vi "FlyWheelCtrl_Example.vi"() -> ()   [LabVIEW 2019]
uses:
  <vilib>/Rock Robotics/WPI/ThirdParty/JAS_Junk/TrajLib/TypeDef/DCMOTOR.CTL
  <vilib>/Rock Robotics/WPI/ThirdParty/JAS_Junk/TrajLib/TypeDef/LINEAR_SYSTEM.ctl
  <vilib>/Analysis/Matrix/Datatypes/RealMatrix.ctl
  <vilib>/Rock Robotics/WPI/ThirdParty/JAS_Junk/TrajLib/TypeDef/FLYWHEEL_SIM.ctl
  <vilib>/Rock Robotics/WPI/ThirdParty/JAS_Junk/TrajLib/TypeDef/LINEAR_SYSTEM_SIM.ctl
  <vilib>/Rock Robotics/WPI/ThirdParty/JAS_Junk/TrajLib/Enum/DCMOTOR_TYPES_ENUM.ctl
  <vilib>/Rock Robotics/WPI/ThirdParty/JAS_Junk/TrajLib/LinearFilter_LP_BW2_Execute.vi
  <vilib>/Rock Robotics/WPI/ThirdParty/JAS_Junk/TrajLib/VI/BoolCmd_Send_Internal.vi
  <vilib>/Rock Robotics/WPI/ThirdParty/JAS_Junk/TrajLib/VI/numCmd_ObtainQueue_OneDbl.vi
  <vilib>/Rock Robotics/WPI/ThirdParty/JAS_Junk/TrajLib/VI/BoolCmd_Recv_Internal.vi
  <vilib>/Rock Robotics/WPI/ThirdParty/JAS_Junk/TrajLib/LinearFilter_ResetToValue.vi
  <vilib>/Rock Robotics/WPI/ThirdParty/JAS_Junk/TrajLib/LinearFilter_Calculate.vi
  <vilib>/Rock Robotics/WPI/ThirdParty/JAS_Junk/TrajLib/VI/BoolCmd_ObtainQueue.vi
  <vilib>/Rock Robotics/WPI/ThirdParty/JAS_Junk/TrajLib/LinearFilter_LowPassBW2.vi
  <vilib>/Rock Robotics/WPI/ThirdParty/JAS_Junk/TrajLib/Trajectory_Library.lvlib
  <vilib>/Analysis/Matrix/NI_Matrix.lvlib
panel:
  in  "Tab Control":T1(tab)
  in  "Speed Setpoint RPM":dbl=2500.0 format="%20.3f"
  out "Motor Current":dbl format="%20.3f"
  out "Battery \nVoltage":dbl format="%20.3f"
  in  "Shoot ball":bool
  out "CO Chart":T2(graph)
  in  "Shooter On/Off":bool
  out "Encoer Speed\nRPM":dbl(slide) scale=0.0..5500.0
  out "Speed RPM":dbl format="%20.3f"
  out "Kalman Filtered\nSpeed RPM":dbl format="%20.3f"
  out "PV Chart":T3(graph)
  out "Controller Error":bool
  out "Motor Volt Dmd (CO)":dbl format="%20.3f"
  out "shoot Start":bool
  out "Shoot Done":bool
  out "Shooter Motor":T4 {"Jr_KgM2" format="%13.5p"; "L_H" format="%13.5p"; "Kt_NMPerAmp" format="%13.5p"; "KvINV_RadPerSecPerVolt" format="%13.5p"; "R_Ohms" format="%13.5p"; "FreeSpeed_RadPerSec" format="%13.5p"; "FreeCurrent_Amps" format="%13.5p"; "StallCurrent_Amps" format="%13.5p"; "StallTorque_NM" format="%13.5p"; "nominalVoltage_Volts" format="%13.5p"}
  out "m_flywheelPlant":T5
  out "m_FlyWheelSim":T7 {"GearBox"."Jr_KgM2" format="%13.5p"; "GearBox"."L_H" format="%13.5p"; "GearBox"."Kt_NMPerAmp" format="%13.5p"; "GearBox"."KvINV_RadPerSecPerVolt" format="%13.5p"; "GearBox"."R_Ohms" format="%13.5p"; "GearBox"."FreeSpeed_RadPerSec" format="%13.5p"; "GearBox"."FreeCurrent_Amps" format="%13.5p"; "GearBox"."StallCurrent_Amps" format="%13.5p"; "GearBox"."StallTorque_NM" format="%13.5p"; "GearBox"."nominalVoltage_Volts" format="%13.5p"}
  out "Shooting A":T6
  out "Shooting B":T6
  # "<States,States>"
  # "<States,Inputs>"
  # "<Outputs,States>"
  # "<Outputs,Inputs>"
  # "<States, 1>"
  # "<Outputs, 1>"
  # "<Inputs, 1>"
  # "<Outputs, 1>"
  # "<States,States>"
  # "<States,Inputs>"
  # "<Outputs,States>"
  # "<Outputs,Inputs>"
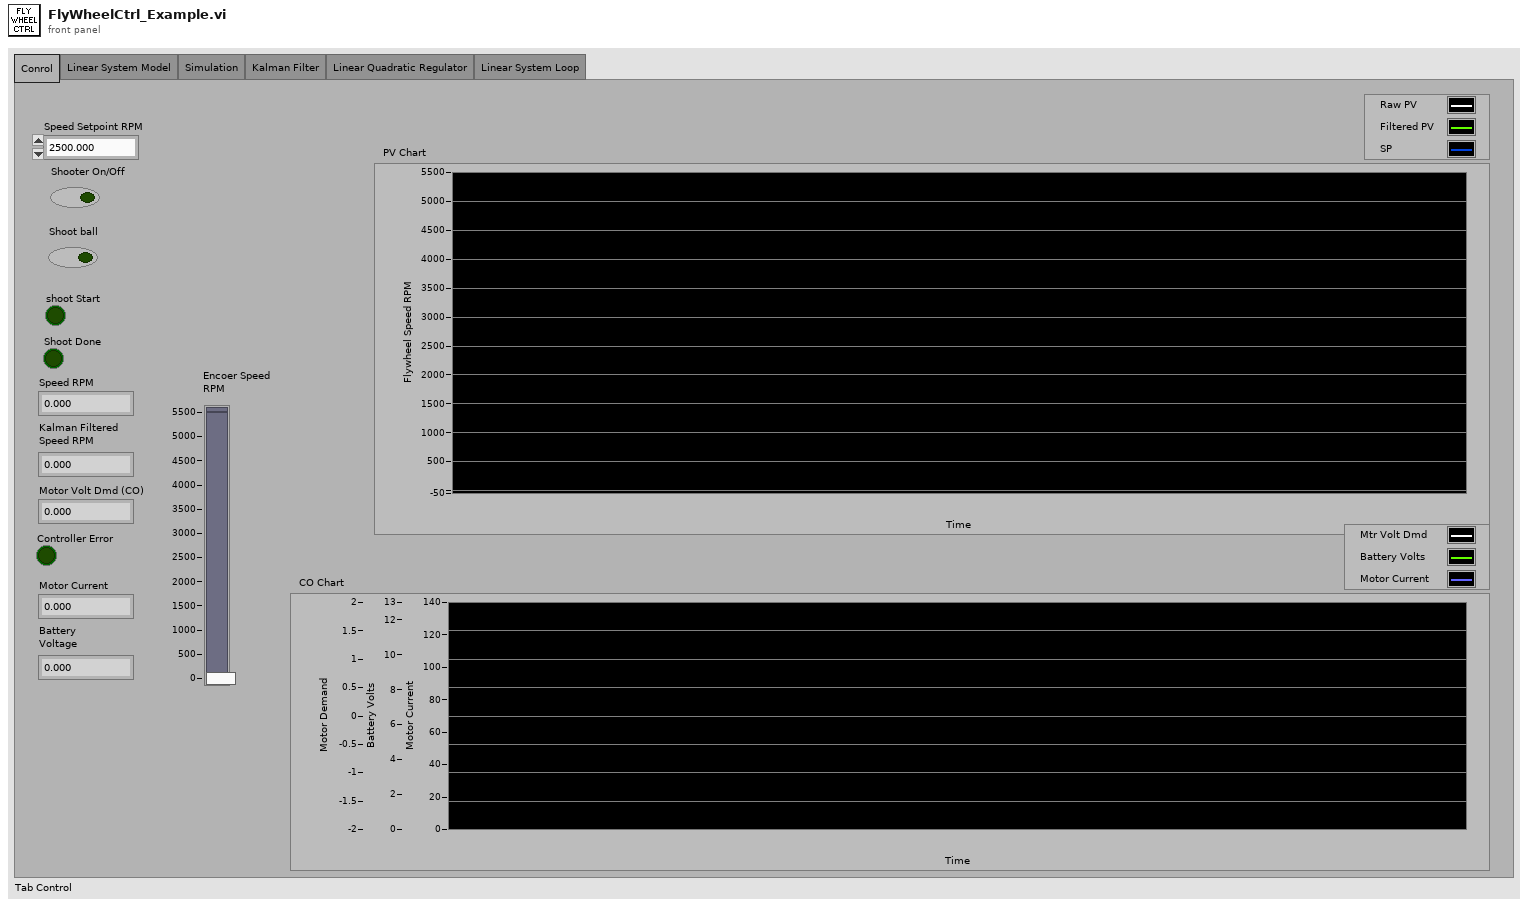
[diagram p1: front panel]
types:
  T1 = enum32{"Conrol", "Linear System Model", "Simulation", "Kalman Filter", "Linear Quadratic Regulator", "Linear System Loop"}
  T2 = cluster{"f":dbl, "Voltage":dbl, "Motor Current":dbl}
  T3 = cluster{"upper limit":dbl, "Real Matrix Element":dbl, "Real Matrix Element":dbl}
  T4 = typedef "Trajectory_Library.lvlib/DCMOTOR.CTL" = cluster{"nominalVoltage_Volts":dbl, "StallTorque_NM":dbl, "StallCurrent_Amps":dbl, "FreeCurrent_Amps":dbl, "FreeSpeed_RadPerSec":dbl, "R_Ohms":dbl, "KvINV_RadPerSecPerVolt":dbl, "Kt_NMPerAmp":dbl, "L_H":dbl, "Jr_KgM2":dbl}
  T5 = typedef "Trajectory_Library.lvlib/LINEAR_SYSTEM.ctl" = cluster{"m_A":T6, "m_B":T6, "m_C":T6, "m_D":T6, "States":i32, "Inputs":i32, "Outputs":i32}
  T6 = typedef "NI_Matrix.lvlib/RealMatrix.ctl" = dbl[][]
  T7 = typedef "Trajectory_Library.lvlib/FLYWHEEL_SIM.ctl" = cluster{"LinearSystemSim":T8, "GearBox":T4, "Gearing":dbl}
  T8 = typedef "Trajectory_Library.lvlib/LINEAR_SYSTEM_SIM.ctl" = cluster{"m_Plant":T5, "m_X":T6, "m_Y":T6, "m_U":T6, "MeasureStdDev":T6}
  T9 = cluster{"RotationsPerMinute":dbl, "Value":dbl, "Value":dbl}
  T10 = typedef "Trajectory_Library.lvlib/DCMOTOR_TYPES_ENUM.ctl" = enum16{"CIM", "AndyMark 9015", "Andy Mark RS 775 125", "Bag", "BaneBots RS 550", "BaneBots RS 775", "Falcon 500", "Mini CIM", "NEO", "NEO 550", "Romi BuiltIn", "Vex 775 Pro", "Snow Blower AM 2235A", "Bosch Seat AM 3493", "Falcon 500 FOC", "Kraken X60", "Kraken X60 FOC", "NEO Vortex"}
  T11 = typedef "Trajectory_Library.lvlib/LINEAR_SYSTEM_ID_FLYWHEEL_MODEL.ctl" = cluster{"DCMOTOR_TYPES":T10, "Num Motors":i32, "Gearing":dbl, "MOI kgm2":dbl}
  T12 = typedef "Trajectory_Library.lvlib/LINEAR_SYSTEM_LOOP_FLYWHEEL_CTRL_PARAMS.CTL" = cluster{"Vel Model Std Dev Rad/Sec":dbl, "Vel Meas Std Dev Rad/Sec":dbl, "Vel Ctrl Tol Rad/Sec":dbl, "Max Ctrl Out V":dbl}
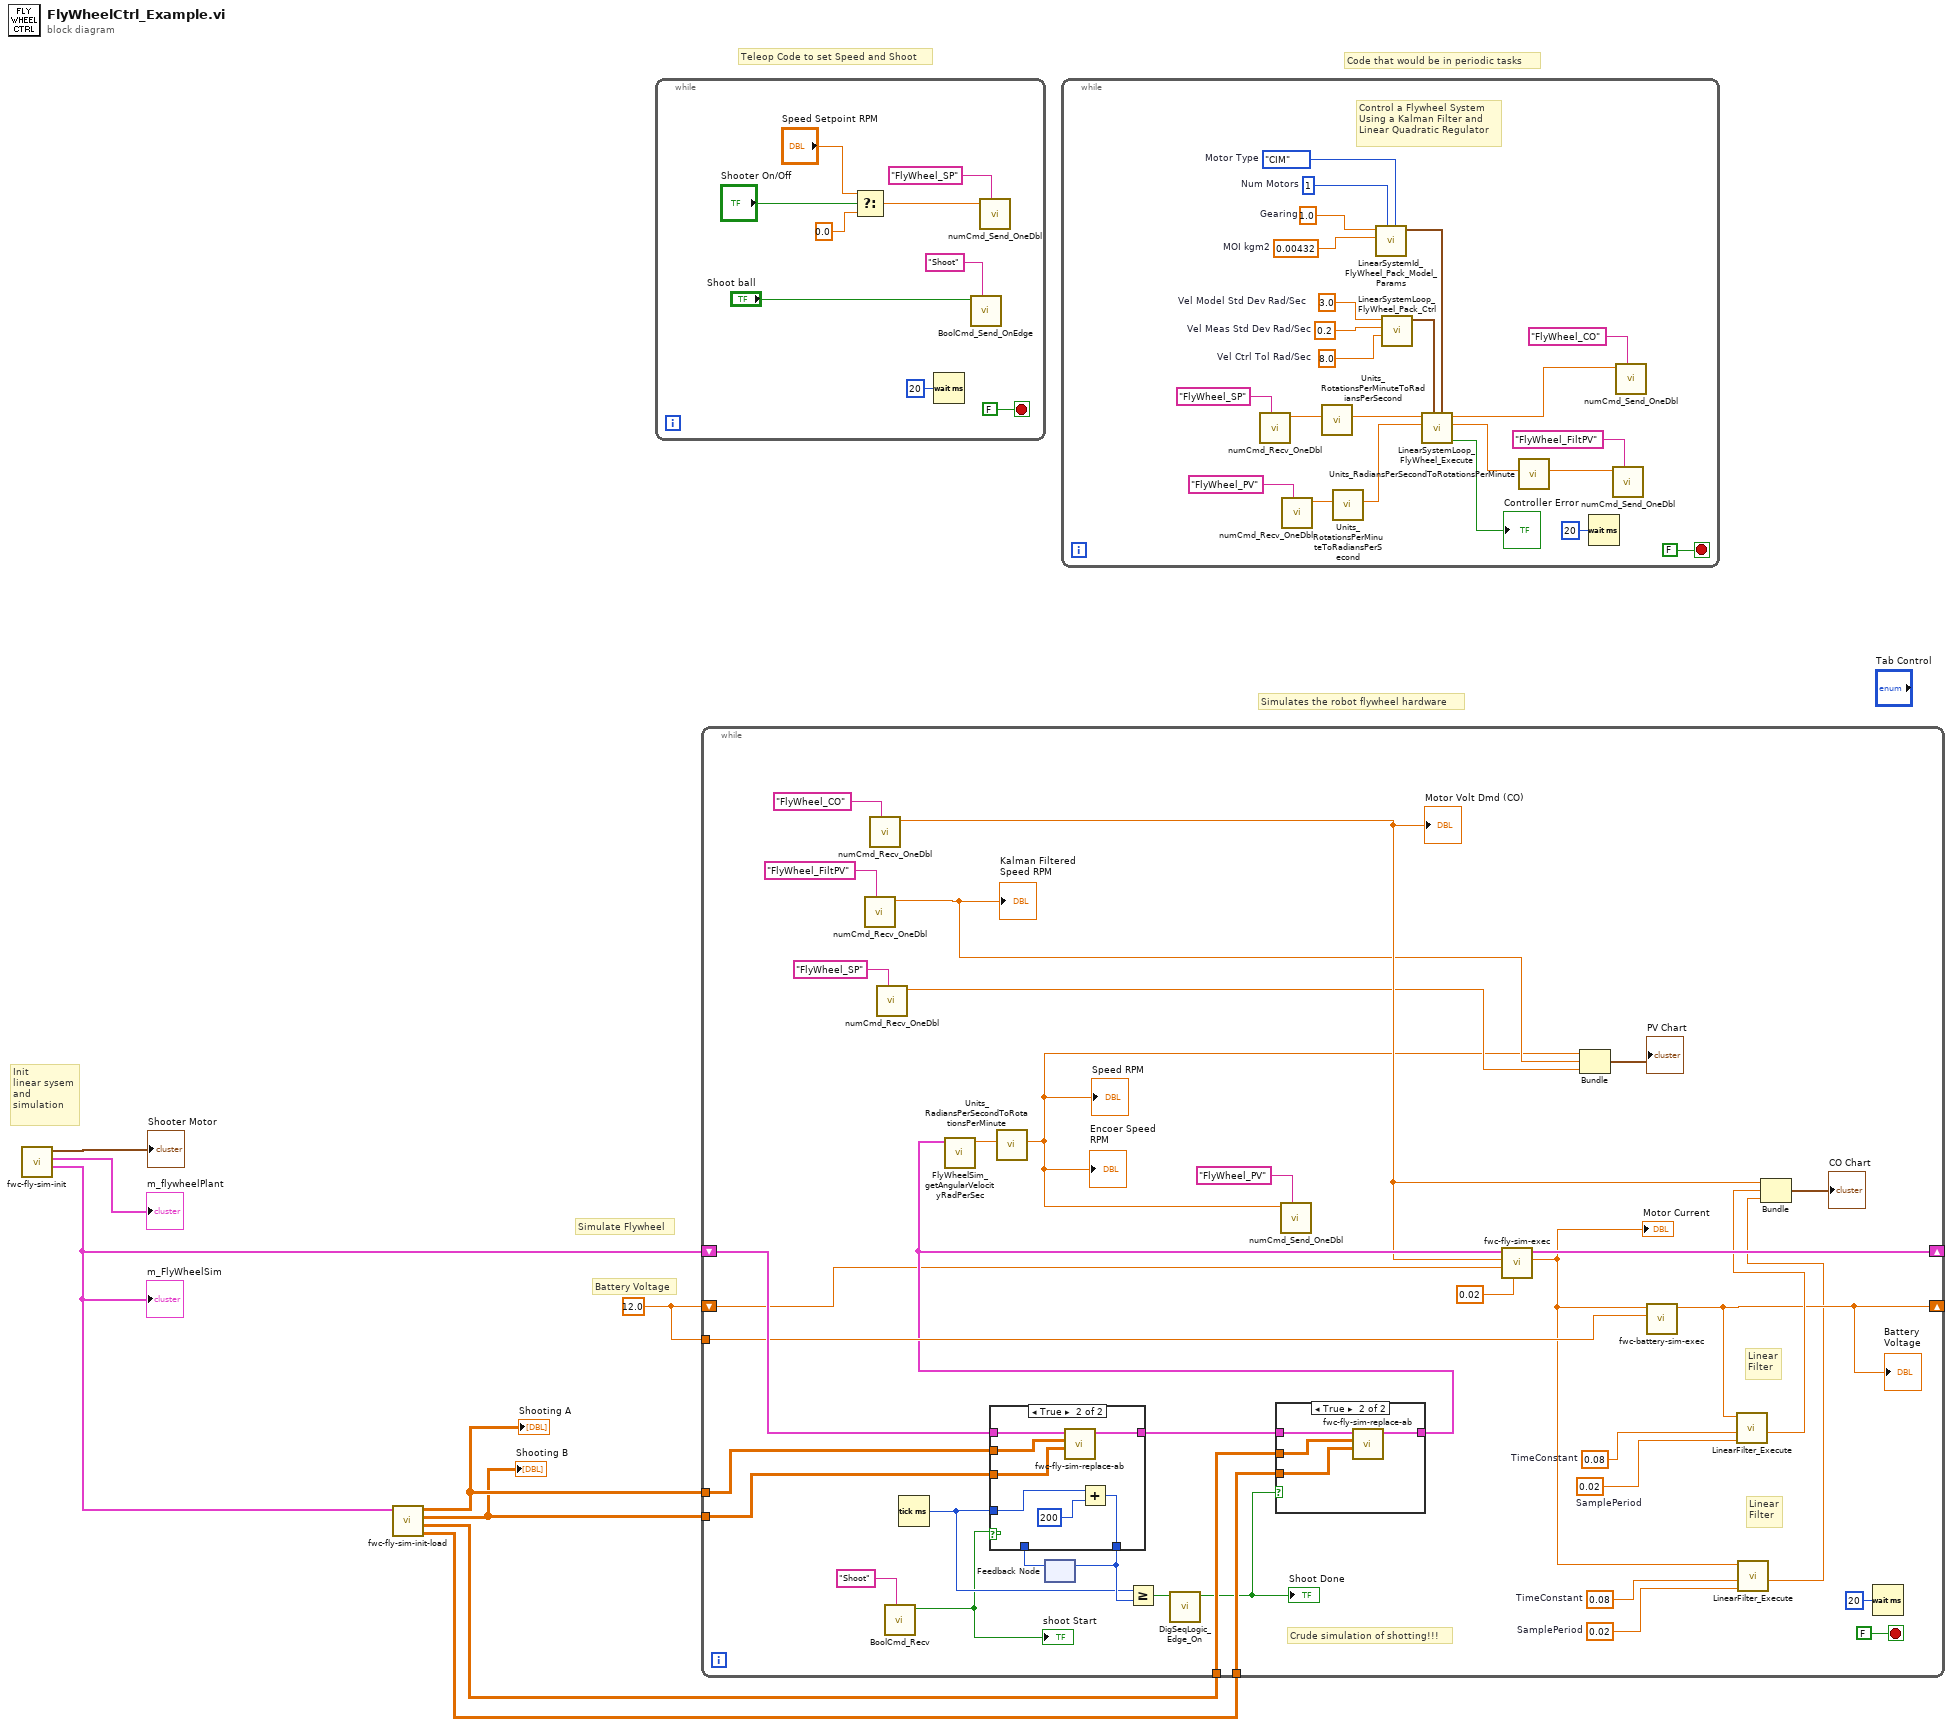
[diagram p0: block diagram]
diagram:
  w7 = 12.0
  # "Teleop Code to set Speed and Shoot"
  # "Code that would be in periodic tasks"
  # "Simulates the robot flywheel hardware"
  # "Init\nlinear sysem\nand \nsimulation"
  # "Simulate Flywheel"
  # "Battery Voltage"
  n1 = call "fwc-fly-sim-init.vi"() -> ("FlyWheelSim"=w6:T7, "Linearsystem"=→"m_flywheelPlant":T5, "DCMOTOR"=→"Shooter Motor":T4)  [unwired: 9 in]
  "m_FlyWheelSim" <- w6
  n2 = call "fwc-fly-sim-init-load.vi"("FlyWheelSim"=w6) -> ("Normal B"=w1:T6, "Normal A"=w2:T6, "Loaded B"=w4:T6, "Loaded A"=w5:T6)  [unwired: 7 in]
  "Shooting A" <- w5
  "Shooting B" <- w4
  n3 = while {
    stop <- FALSE stop-if-true
    n4 = Select(t="Speed Setpoint RPM", s="Shooter On/Off", f=0.0) -> (s? t:f=w14:dbl)
    n5 = Wait (ms)(milliseconds to wait=u32 20) -> ()  [unwired: 1 out]
    n6 = call <vilib>:"BoolCmd_Send_OnEdge.vi"("Command Name"="Shoot", "Value"="Shoot ball") -> ()  [unwired: 9 in, 1 out]
    n7 = call <vilib>:"numCmd_Send_OneDbl.vi"("Command Name"="FlyWheel_SP", "Value"=w14) -> ()  [unwired: 9 in, 1 out]
  }
  n8 = while {
    shift-right: [w53] -> _
    shift-left: w6 -> [w51]
    shift-right: [w35] -> _
    shift-left: w7 -> [w39]
    tunnel: w7 -> [w43]
    tunnel: w2 -> [w49]
    tunnel: w1 -> [w48]
    tunnel: w5 -> [w47]
    tunnel: w4 -> [w46]
    stop <- FALSE stop-if-true
    w37 = 0.02  # SamplePeriod
    w19 = 0.08  # TimeConstant
    w38 = 0.02  # SamplePeriod
    w18 = 0.08  # TimeConstant
    # "Linear\nFilter"
    # "Linear\nFilter"
    # "Crude simulation of shotting!!!"
    n9 = call <vilib>:"numCmd_Recv_OneDbl.vi"("Command Name"="FlyWheel_FiltPV") -> ("Value"=w29:dbl)  [unwired: 8 in, 2 out]
    "Kalman Filtered\nSpeed RPM" <- w29
    n10 = call <vilib>:"numCmd_Recv_OneDbl.vi"("Command Name"="FlyWheel_CO") -> ("Value"=w31:dbl)  [unwired: 8 in, 2 out]
    "Motor Volt Dmd (CO)" <- w31
    n11 = call <vilib>:"numCmd_Recv_OneDbl.vi"("Command Name"="FlyWheel_SP") -> ("Value"=w27:dbl)  [unwired: 8 in, 2 out]
    n12 = call <vilib>:"BoolCmd_Recv.vi"("Command Name"="Shoot") -> ("New Request"=w20:bool)  [unwired: 9 in, 1 out]
    "shoot Start" <- w20
    n13 = Tick Count (ms)() -> (millisecond timer value=w42:u32)
    n14 = feedback #1() -> (w44:u32)  [unwired: 1 in]
    n15 = case shown="True" w20 {
      tunnel: w51 -> [w63 w68]
      tunnel: [w63 w67] -> w50
      tunnel: w47 -> [_ w66]
      tunnel: w46 -> [_ w65]
      tunnel: [w62 w69] -> w45
      tunnel: w44 -> [w62 _]
      tunnel: w42 -> [_ w64]
      frame False {
      }
      frame True {
        n16 = call "fwc-fly-sim-replace-ab.vi"("B"=w65, "A"=w66, "in FlyWheelSim"=w68) -> ("out FlyWheelSim"=w67:T7)  [unwired: 8 in]
        n17 = Add(x=w64, y=u32 200) -> (x+y=w69:u32)
      }
    }
    n18 = feedback-in #1(w45) -> ()
    n19 = Greater Or Equal?(x=w42, y=w45) -> (x >= y?=w22:bool)
    n20 = call <vilib>:"DigSeqLogic_Edge_On.vi"("Input"=w22) -> ("On Edge"=w23:bool)  [unwired: 10 in]
    "Shoot Done" <- w23
    n21 = case shown="True" w23 {
      tunnel: w50 -> [w57 w61]
      tunnel: [w57 w60] -> w40
      tunnel: w49 -> [_ w59]
      tunnel: w48 -> [_ w58]
      frame False {
      }
      frame True {
        n22 = call "fwc-fly-sim-replace-ab.vi"("B"=w58, "A"=w59, "in FlyWheelSim"=w61) -> ("out FlyWheelSim"=w60:T7)  [unwired: 8 in]
      }
    }
    n23 = call <vilib>:"FlyWheelSim_getAngularVelocityRadPerSec.vi"("FlyWheelSim"=w40) -> ("Velocity_RadPerSec"=w26:dbl)  [unwired: 10 in]
    n24 = call <vilib>:"Units_RadiansPerSecondToRotationsPerMinute.vi"("RadiansPerSecond"=w26) -> ("RotationsPerMinute"=w24:dbl)  [unwired: 10 in]
    "Encoer Speed\nRPM" <- w24
    "Speed RPM" <- w24
    n25 = call <vilib>:"numCmd_Send_OneDbl.vi"("Command Name"="FlyWheel_PV", "Value"=w24) -> ()  [unwired: 9 in, 1 out]
    n26 = call "fwc-fly-sim-exec.vi"("dT_Seconds"=0.02, "Battery Voltage"=w39, "Motor Dmd (CO)"=w31, "in FlyWheelSim"=w40) -> ("Motor Current"=w34:dbl, "out FlyWheelSim"=w53:T7)  [unwired: 6 in]
    "Motor Current" <- w34
    n27 = Bundle("RotationsPerMinute"=w24, "Value"=w29, "Value"=w27) -> (→"PV Chart":T9)  [unwired: 1 in]
    n28 = call "fwc-battery-sim-exec.vi"("Numeric"=w43, "Motor Current"=w34) -> ("Voltage"=w35:dbl)  [unwired: 9 in]
    "Battery \nVoltage" <- w35
    n29 = call-poly <vilib>:"LinearFilter_Execute.vi"("SamplePeriod"=w38, "TimeConstant"=w18, "Input"=w35) -> ("Output"=w36:dbl)  [unwired: 8 in]
    n30 = call-poly <vilib>:"LinearFilter_Execute.vi"("SamplePeriod"=w37, "TimeConstant"=w19, "Input"=w34) -> ("Output"=w33:dbl)  [unwired: 8 in]
    n31 = Bundle("Value"=w31, "Output"=w36, "Output"=w33) -> (→"CO Chart":cluster{"Value":dbl, "Output":dbl, "Output":dbl})  [unwired: 1 in]
    n32 = Wait (ms)(milliseconds to wait=u32 20) -> ()  [unwired: 1 out]
  }
  n33 = while {
    stop <- FALSE stop-if-true
    w83 = 3.0  # Vel Model Std Dev Rad/Sec
    w84 = 0.2  # Vel Meas Std Dev Rad/Sec
    w85 = 8.0  # Vel Ctrl Tol Rad/Sec
    w90 = 1.0  # Gearing
    w91 = 0.00432  # MOI kgm2
    w92 = 1  # Num Motors
    w93 = DCMOTOR_TYPES_ENUM."CIM"  # Motor Type
    # "Control a Flywheel System\nUsing a Kalman Filter and \nLinear Quadratic Regulator"
    n34 = call <vilib>:"numCmd_Recv_OneDbl.vi"("Command Name"="FlyWheel_SP") -> ("Value"=w77:dbl)  [unwired: 8 in, 2 out]
    n35 = call <vilib>:"numCmd_Recv_OneDbl.vi"("Command Name"="FlyWheel_PV") -> ("Value"=w81:dbl)  [unwired: 8 in, 2 out]
    n36 = call <vilib>:"Units_RotationsPerMinuteToRadiansPerSecond.vi"("RotationsPerMinute"=w77) -> ("RadiansPerSecond"=w79:dbl)  [unwired: 10 in]
    n37 = call <vilib>:"Units_RotationsPerMinuteToRadiansPerSecond.vi"("RotationsPerMinute"=w81) -> ("RadiansPerSecond"=w80:dbl)  [unwired: 10 in]
    n38 = call <vilib>:"LinearSystemId_FlyWheel_Pack_Model_Params.vi"("DCMOTOR_TYPES"=w93, "Num Motors"=w92, "MOI kgm2"=w91, "Gearing"=w90) -> ("LinearSystem_ID_FlyWheel_Model"=w87:T11)  [unwired: 7 in]
    n39 = call <vilib>:"LinearSystemLoop_FlyWheel_Pack_Ctrl.vi"("Vel Ctrl Tol Rad/Sec"=w85, "Vel Meas Std Dev Rad/Sec"=w84, "Vel Model Std Dev Rad/Sec"=w83) -> ("LinearSystemLoop_FlyWheel_Ctrl_Params"=w86:T12)  [unwired: 8 in]
    n40 = call <vilib>:"LinearSystemLoop_FlyWheel_Execute.vi"("FlyWheelSim_Model _Params"=w87, "LinearSystem_FlyWheel_Ctrl_Params"=w86, "Velocity (Rad/Sec)\n(PV)"=w80, "Velocity (Rad/Sec)\nSetpoint (SP)"=w79) -> ("Error"=→"Controller Error":bool, "Kalman FIltered\nVelocity (PV)"=w72:dbl, "Motor Dmd"=w75:dbl)  [unwired: 5 in]
    n41 = call <vilib>:"Units_RadiansPerSecondToRotationsPerMinute.vi"("RadiansPerSecond"=w72) -> ("RotationsPerMinute"=w73:dbl)  [unwired: 10 in]
    n42 = Wait (ms)(milliseconds to wait=u32 20) -> ()  [unwired: 1 out]
    n43 = call <vilib>:"numCmd_Send_OneDbl.vi"("Command Name"="FlyWheel_FiltPV", "Value"=w73) -> ()  [unwired: 9 in, 1 out]
    n44 = call <vilib>:"numCmd_Send_OneDbl.vi"("Command Name"="FlyWheel_CO", "Value"=w75) -> ()  [unwired: 9 in, 1 out]
  }
